vi "Actor Core.vi"(8 "error in":cluster{"状态":bool, "代码":i32, "源":string} caption="错误输入", 11 "MapDisplayer":refnum<class "Map.lvclass">) -> (0 "error out":cluster{"状态":bool, "代码":i32, "源":string} caption="错误输出", 3 "操作者输出":refnum<class "Actor.lvclass">)   [LabVIEW 2014, in "Map.lvlib" / "Map.lvclass"]
doc: "Actor Core.vi包含操作者的主要消息处理循环。操作者通常位于该循环中，在各种消息到达时对消息进行处理。如Do.vi消息返回任何错误，该循环将停止运行，错误代码43将被作为“无错误停止”的标准信号发送给调用方。如需更改上述行为，可在子孙类的Handle Error.vi中对该部分逻辑进行重写。"
uses:
  Map.lvclass
  <vilib>/ActorFramework/Actor/Actor.lvclass
  MapBuilder/Robot_Position.ctl
  <vilib>/ActorFramework/Actor/Actor.lvclass/Actor.ctl
  Map.lvclass/Map.ctl
  <vilib>/ActorFramework/Message Enqueuer/Message Enqueuer.lvclass/Message Enqueuer.ctl
  <vilib>/ActorFramework/Message Enqueuer/Enqueue.vi
  <vilib>/ActorFramework/Message Priority Queue/Priority Enqueue.vi
  <vilib>/ActorFramework/Message Enqueuer/Message Enqueuer.lvclass
  Wrapper_lib/zsActor/ActorWrapper.lvclass
panel:
  out "vel_cal":cluster{"rot_z":dbl, "lin_x":dbl} {"lin_x" scale=0.0..0.6; "rot_z" scale=0.6..-0.6}
  in  "MapPosition":T1
  in  "robot position":T2
  out "平面俯视图":T3(plugin-control)
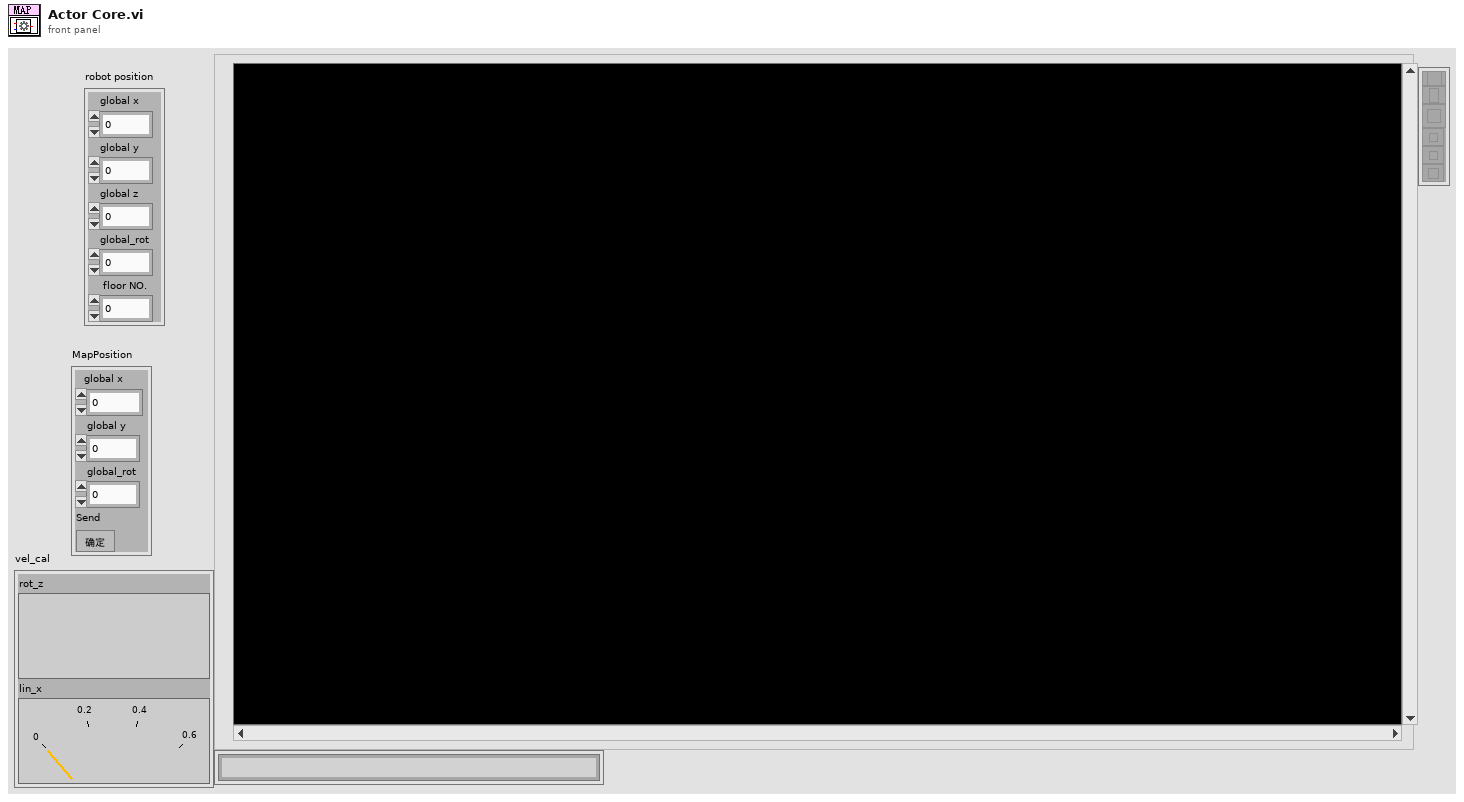
[diagram p1: front panel]
types:
  T1 = cluster{"global x":dbl, "global y":dbl, "global_rot":dbl, "Send":bool}
  T2 = typedef "Robot_Position.ctl" = cluster{"global x":dbl, "global y":dbl, "global z":dbl, "global_rot":dbl, " floor NO.":dbl}
  T3 = typedef "IMAQ Image.ctl" = refnum<image>
  T4 = typedef "NI_Matrix.lvlib/RealMatrix.ctl" = dbl[][]
  T5 = cluster{"District Name":string, "Alias":string, "District Type":string, "Floor NO.":string, "Data Matrix":T4, "Path array":string[], "Path Coodinate":T4}[]
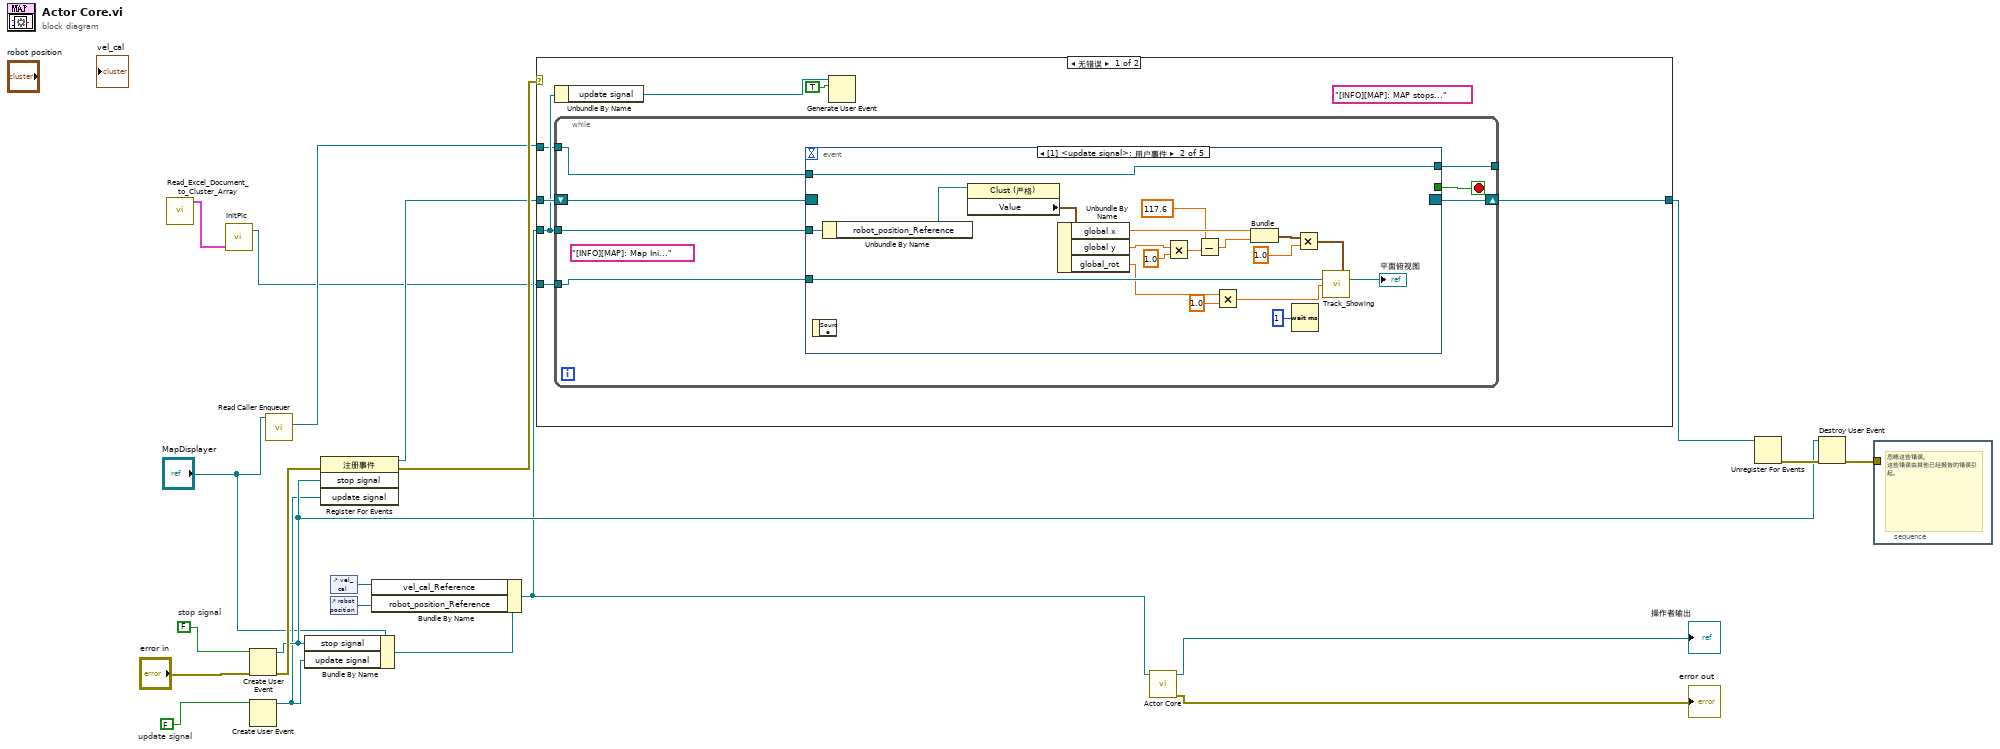
[diagram p0: block diagram]
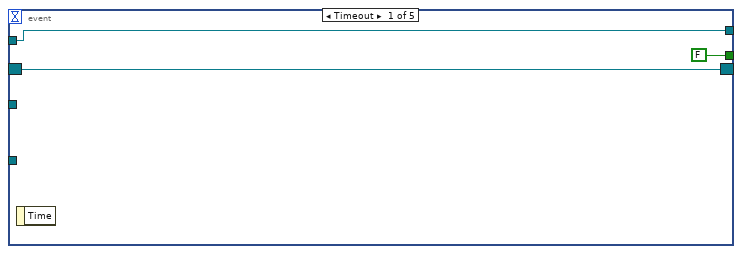
[diagram p2: hidden frame]
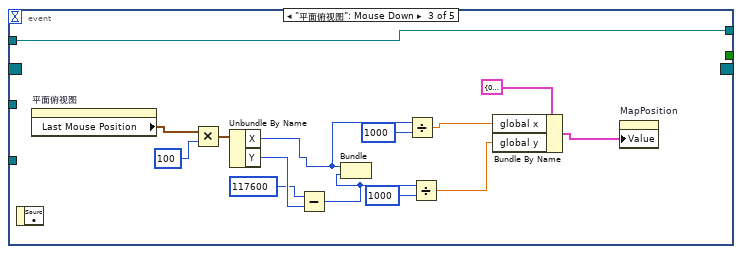
[diagram p3: hidden frame]
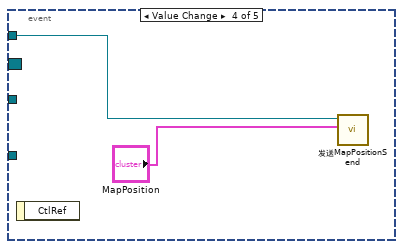
[diagram p4: hidden frame]
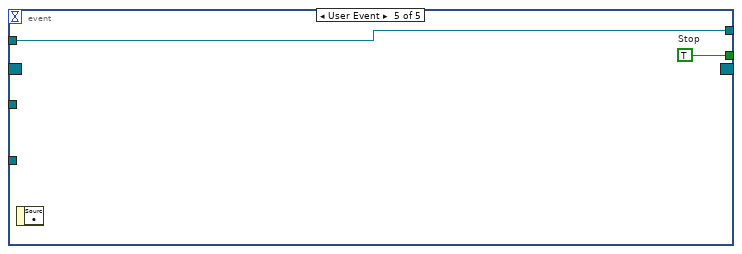
[diagram p5: hidden frame]
diagram:
  w8 = FALSE  # update signal
  w16 = FALSE  # stop signal
  n1 = call "Read_Excel_Document_to_Cluster_Array.vi"() -> ("Cluster of 7 Type Data_4F"=w1:T5)  [unwired: 7 in, 4 out]
  n2 = call "InitPic.vi"("Cluster of 7 Type Data"=w1) -> ("Image Out 2"=w4:T3)  [unwired: 3 in]
  n3 = Create User Event(user event datatype=w16, error in="error in") -> (user event=w10:refnum<user-event>, error out=w17:errorcluster)
  n4 = Create User Event(user event datatype=w8) -> (user event=w7:refnum<user-event>)  [unwired: 1 in, 1 out]
  n5 = call <vilib>:"Read Caller Enqueuer.vi"("Actor"="MapDisplayer") -> ("Caller Enqueuer"=w5:refnum<class "Message Enqueuer.lvclass">)  [unwired: 10 in]
  n6 = Bundle By Name(cluster="MapDisplayer", "stop signal"=w10, "update signal"=w7) -> (w18:refnum<class "Map.lvclass">)
  n7 = register-events(error in=w17, w10, w7) -> (reference out=w14:refnum<event-registration>, error out=w15:errorcluster)  [unwired: 1 in]
  n8 = control-ref of="vel_cal"() -> (w2:refnum<vi>)
  n9 = control-ref of="robot position"() -> (w3:refnum<vi>)
  n10 = Bundle By Name(cluster=w18, "vel_cal_Reference"=w2, "robot_position_Reference"=w3) -> (w9:refnum<class "Map.lvclass">)
  n11 = case shown="无错误" w15 {
    tunnel: w14 -> [w28 w76]
    tunnel: [w27 w76] -> w13
    tunnel: w9 -> [w26 _]
    tunnel: w5 -> [w23 _]
    tunnel: w4 -> [w22 _]
    frame No Error {
      (unwired) "[INFO][MAP]: MAP stops..." ("Event Text")
      n12 = Unbundle By Name(w26) -> ("update signal"=w25:refnum<user-event>)
      n13 = while {
        shift-right: [w34] -> w27
        shift-left: w28 -> [w35]
        tunnel: w26 -> [w32]
        tunnel: w23 -> [w30]
        tunnel: w22 -> [w31]
        tunnel: [w29] -> _
        stop <- w33 stop-if-true
        (unwired) "[INFO][MAP]: Map Ini..." ("Event Text")
        n14 = event shown="[1] <update signal>: 用户事件" {
          selector: w35 -> [w38 _ _ _ _]
          dyn-events: [w38 _ _ _ _] -> w34
          timeout: _ -> [_ _ _ _ _]
          tunnel: [FALSE ("Stop") _ _ _ w75] -> w33
          tunnel: w32 -> [_ w55 _ _ _]
          tunnel: w30 -> [w36 w47 w71 w73 w74]
          tunnel: w31 -> [_ w50 _ _ _]
          tunnel: [w36 w47 w71 _ w74] -> w29
          event Timeout {
            n15 = event-data() -> ()  [unwired: 1 in, 1 out]
          }
          event User Event {
            n16 = event-data() -> ()  [unwired: 1 in, 1 out]
            n17 = Unbundle By Name(w55) -> ("robot_position_Reference"=w56:refnum<vi>)
            n18 = property class="Clust (严格)"(reference=w56) -> ("Value"=w57:T2)  [unwired: 1 in, 2 out]
            n19 = Unbundle By Name(w57) -> ("global x"=w51:dbl, "global y"=w43:dbl, "global_rot"=w45:dbl)
            n20 = Multiply(x=w43, y=1.0) -> (x*y=w42:dbl)
            n21 = Subtract(x=117.6, y=w42) -> (x-y=w40:dbl)
            n22 = Multiply(x=w45, y=1.0) -> (x*y=w46:dbl)
            n23 = Bundle("global x"=w51, w40) -> (w54:cluster{"global x":dbl, dbl})  [unwired: 1 in]
            n24 = Wait (ms)(milliseconds to wait=u32 1 ("等待时间（毫秒）")) -> ()  [unwired: 1 out]
            n25 = Multiply(x=w54, y=1.0) -> (x*y=w52:cluster{"global x":dbl, dbl})
            n26 = call "Track_Showing.vi"("NewNodeM"=w52, "Image In 2"=w50, "数值"=w46) -> ("Image Out 2"=→"平面俯视图":T3)  [unwired: 12 in]
          }
          event "平面俯视图": Mouse Down {
            n27 = event-data() -> ()  [unwired: 1 in, 1 out]
            n28 = property on="平面俯视图" class="ImageControl"() -> ("Last Mouse Position"=w70:cluster{"X":i32, "Y":i32})  [unwired: 2 in, 2 out]
            n29 = Multiply(x=w70, y=100) -> (x*y=w68:cluster{"X":i32, "Y":i32})
            n30 = Unbundle By Name(w68) -> ("X"=w65:i32, "Y"=w60:i32)
            n31 = Subtract(x=117600, y=w60) -> (x-y=w58:i32)
            n32 = Bundle("X"=w65, w58) -> ()  [unwired: 1 in, 1 out]
            n33 = Divide(x=w65, y=1000) -> (x/y=w62:dbl)
            n34 = Divide(x=w58, y=1000) -> (x/y=w61:dbl)
            n35 = Bundle By Name(cluster=T1 {"global x"=0.0, "global y"=0.0, "global_rot"=0.0, "Send"=FALSE} ("MapPosition 2"), "global x"=w62, "global y"=w61) -> (w66:T1)
            n36 = property on="MapPosition" class="Clust"("Value"=w66) -> ()  [unwired: 2 in, 2 out]
          }
          event "MapPosition.Send": Value Change {
            n37 = event-data() -> ()  [unwired: 1 in, 1 out]
            n38 = call "发送MapPositionSend.vi"("MapPosition"="MapPosition", "消息待入队列"=w73) -> ()  [unwired: 8 in, 2 out]
          }
          event User Event {
            w75 = TRUE  # Stop
            n39 = event-data() -> ()  [unwired: 1 in, 1 out]
          }
        }
      }
      n40 = Generate User Event(user event=w25, event data cluster=TRUE ("事件数据")) -> ()  [unwired: 2 in, 2 out]
    }
    frame Error {
    }
  }
  n41 = call-parent "Actor Core.vi"("Actor in"=w9) -> ("error out"=→"error out":errorcluster, "Actor out"=→"操作者输出":refnum<class "Actor.lvclass">)  [unwired: 9 in]
  n42 = Unregister For Events(event registration refnum=w13) -> (error out=w12:errorcluster)  [unwired: 1 in]
  n43 = Destroy User Event(user event=w10, error in=w12) -> (error out=w11:errorcluster)
  n44 = stacked-sequence {
    tunnel: w11 -> [_]
    frame #0 {
      # "忽略这些错误。\n这些错误由其他已经报告的错误引起。"
    }
  }
